vi "BB Writer from Refnum.vi"(3 "BB Writer Refnum":T1 {"refnum" format="%.0x"}) -> (5 "BB Writer U64":u64)   [LabVIEW 2021, in "Iceoryx.lvlib"]
uses:
  Iceoryx.lvlib
  Typedef/BB Writer Refnum.ctl
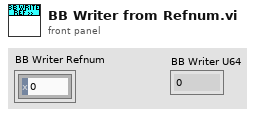
[diagram p1: front panel]
types:
  T1 = typedef "Iceoryx.lvlib/BB Writer Refnum.ctl" = cluster{"refnum":u64, "BB Writer":enum8{"bb_writer"}}
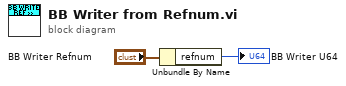
[diagram p0: block diagram]
diagram:
  n1 = Unbundle By Name("BB Writer Refnum") -> ("refnum"=→"BB Writer U64":u64)
